vi "Environment Variable for Main venv--constant.vi"() -> (3 "Environment Variable for Main venv":string="py2vi_tool_venv")   [LabVIEW 2026]
doc: "This constant describes the environment variable that defines the path to the virtual environment that is used by the tool."
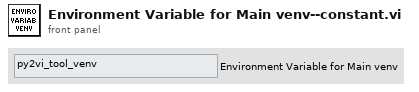
[diagram p1: front panel]
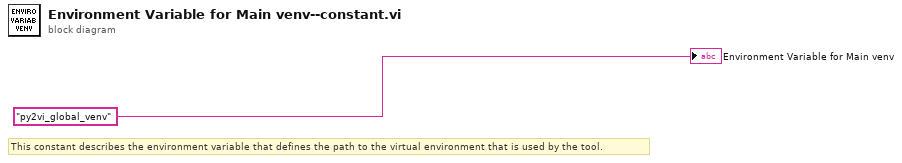
[diagram p0: block diagram]
diagram:
  # "This constant describes the environment variable that defines the path to the virtual environment that is used by the tool."
  "Environment Variable for Main venv" <- "py2vi_global_venv"
